vi "current_pulse_train.vi"() -> ()   [LabVIEW 2025, in "tSNIP.lvlib"]
uses:
  tSNIP.lvlib
panel:
  out "error out":errorcluster
  in  "error in":errorcluster
  in  "Current Type":enum32{"Constant", "Staircase"}(tab)
  in  "Current Amplitude":cluster{"Value":dbl, "Units":dbl}={"Value"=0.0, "Units"=0.001} {"Units" items=["mA"=0.001, "A"=1.0]}
  in  "Current Step":cluster{"Value":dbl, "Units":dbl}={"Value"=0.0, "Units"=0.001} {"Units" items=["mA"=0.001, "A"=1.0]}
  out "Current Waveform":waveform(dbl)(graph)
  in  "Duty Cycle":T1={"ON"={"Units"=1.0, "Value"=10.0}, "OFF"={"Units"=1, "Value"=10.0}} {"OFF"."Units" items=["s"=1, "min"=60, "hr"=3600]; "ON"."Units" items=["ms"=0.001, "s"=1.0, "min"=60.0, "hr"=3600.0]}
  in  "Cycles":u64=1 min=1
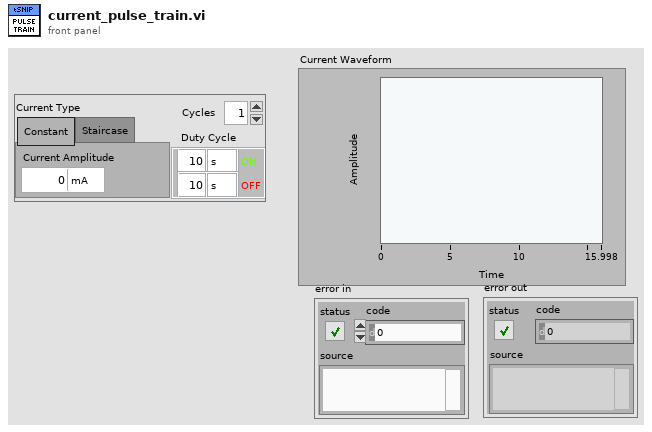
[diagram p1: front panel]
types:
  T1 = cluster{"ON":cluster{"Units":dbl, "Value":dbl}, "OFF":cluster{"Units":u16, "Value":dbl}}
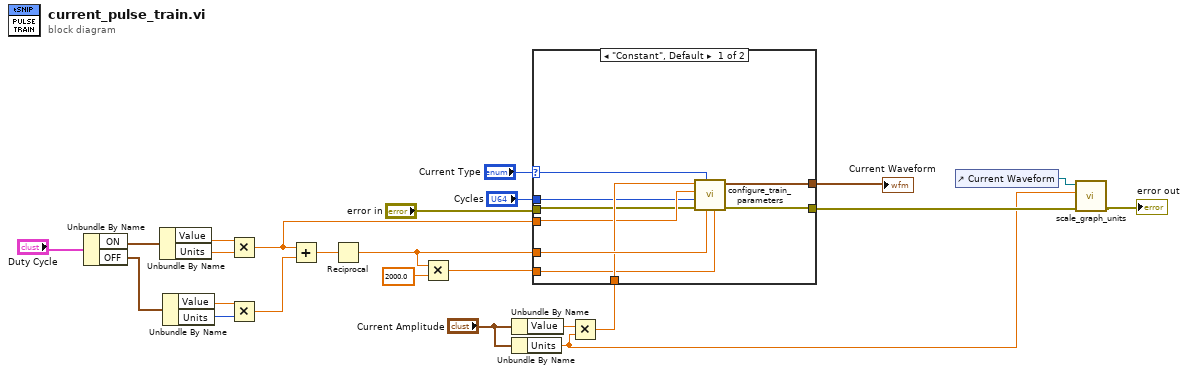
[diagram p0: block diagram]
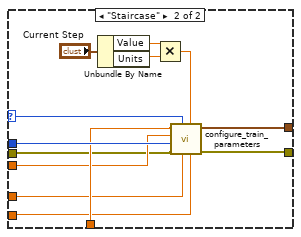
[diagram p2: hidden frame]
diagram:
  n1 = Unbundle By Name("Duty Cycle") -> ("ON"=w22:cluster{"Units":dbl, "Value":dbl}, "OFF"=w14:cluster{"Units":u16, "Value":dbl})
  n2 = Unbundle By Name(w22) -> ("Value"=w23:dbl, "Units"=w16:dbl)
  n3 = Unbundle By Name(w14) -> ("Value"=w24:dbl, "Units"=w15:u16)
  n4 = Multiply(x=w23, y=w16) -> (x*y=w10:dbl)
  n5 = Multiply(x=w24, y=w15) -> (x*y=w20:dbl)
  n6 = Add(x=w10, y=w20) -> (x+y=w11:dbl)
  n7 = Reciprocal(x=w11) -> (1/x=w7:dbl)
  n8 = Multiply(x=w7, y=2000.0) -> (x*y=w6:dbl)
  n9 = Unbundle By Name("Current Amplitude") -> ("Value"=w18:dbl)
  n10 = Unbundle By Name("Current Amplitude") -> ("Units"=w3:dbl)
  n11 = Multiply(x=w18, y=w3) -> (x*y=w12:dbl)
  n12 = case shown="\"Constant\", Default" "Current Type" {
    selector: "Current Type" -> [w29 w41]
    tunnel: "Cycles" -> [w30 w45]
    tunnel: w12 -> [w32 w40]
    tunnel: w7 -> [w33 w39]
    tunnel: w10 -> [w31 w38]
    tunnel: [w28 w37] -> w9
    tunnel: w6 -> [w27 w36]
    tunnel: [w26 w35] -> w4
    tunnel: "error in" -> [w25 w34]
    frame "Constant", Default {
      n13 = call "configure_train_parameters.vi"("Fs"=w27, "Frequency"=w33, "Current Type"=w29, "error in"=w25, "NumCycles"=w30, "Pulse width"=w31, "Amplitude"=w32) -> ("error out"=w26:errorcluster, "Output train"=w28:waveform(dbl))  [unwired: 3 in]
    }
    frame "Staircase" {
      n14 = Unbundle By Name("Current Step") -> ("Value"=w44:dbl, "Units"=w43:dbl)
      n15 = Multiply(x=w44, y=w43) -> (x*y=w42:dbl)
      n16 = call "configure_train_parameters.vi"("Fs"=w36, "Amplitude Step"=w42, "Frequency"=w39, "Current Type"=w41, "error in"=w34, "NumCycles"=w45, "Pulse width"=w38, "Amplitude"=w40) -> ("error out"=w35:errorcluster, "Output train"=w37:waveform(dbl))  [unwired: 2 in]
    }
  }
  "Current Waveform" <- w9
  n17 = control-ref of="Current Waveform"() -> (w1:refnum<vi>)
  n18 = call "scale_graph_units.vi"("error in"=w4, "y-units"=w3, "reference in"=w1) -> ("error out"=→"error out":errorcluster)  [unwired: 6 in, 1 out]
